vi "Host_Close.vi"(8 "error in (no error)":errorcluster={"status"=FALSE, "code"=0, "source"="\"\""}, 10 "close policy":string, 11 "Host refs":string) -> (0 "error out":errorcluster={"status"=FALSE, "code"=0, "source"="\"\""}, 2 "status ok":bool, 3 "Error/status":string)   [LabVIEW 2026]
doc: "INTENT: Stop Host services. LOGIC: Stop UI senders, close connections, drain mandatory audit events and release references."
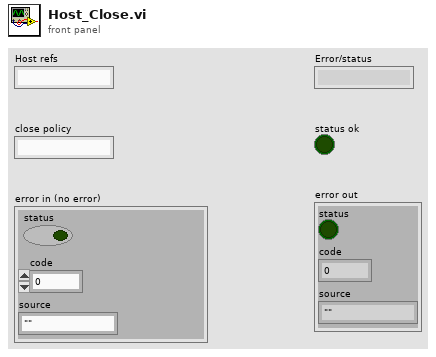
[diagram p1: front panel]
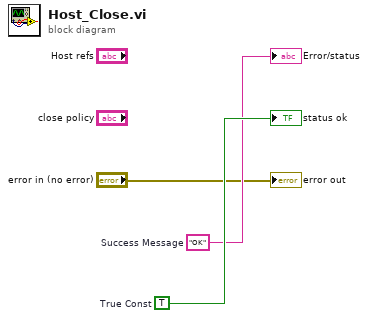
[diagram p0: block diagram]
diagram:
  w3 = TRUE  # True Const
  w2 = "OK"  # Success Message
  "Error/status" <- w2
  "status ok" <- w3
  "error out" <- "error in (no error)"
